vi "Register gRPC Methods.vi"(8 "error in (no error)":errorcluster, 11 "gRPC service in":refnum<class "CanReaderNixnet.lvclass">) -> (0 "error out":errorcluster, 3 "gRPC service out":refnum<class "CanReaderNixnet.lvclass">)   [LabVIEW 2021, in "CanReaderNixnet_server.lvlib" / "CanReaderNixnet.lvclass"]
uses:
  CanReaderNixnet.lvclass
  typeDefs/Server Internal UEs.ctl
  typeDefs/Server Internal Message.ctl
  typeDefs/Server gRPC UEs.ctl
  <vilib>/gRPC/LabVIEW gRPC Library/Server API/typeDefs/gRPCId Cluster.ctl
  <vilib>/gRPC/LabVIEW gRPC Library/Shared/grpcId.ctl
  CanReaderNixnet.lvclass/CanReaderNixnet.ctl
  <vilib>/gRPC/LabVIEW gRPC Library/grpc-lvsupport-release.lvlib
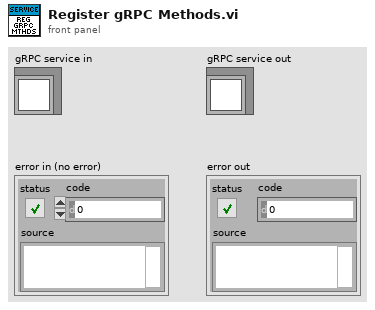
[diagram p1: front panel]
types:
  T1 = typedef "CanReaderNixnet_server.lvlib/CanReaderNixnet.lvclass/Server gRPC UEs.ctl" = cluster{"CanReaderNixnet GetDevices gRPC UE":refnum<user-event>, "CanReaderNixnet GetStatistics gRPC UE":refnum<user-event>, "CanReaderNixnet SetInterfaceBlink gRPC UE":refnum<user-event>, "CanReaderNixnet GetCANStatus gRPC UE":refnum<user-event>}
  T2 = typedef "CanReaderNixnet_server.lvlib/CanReaderNixnet.lvclass/Server Internal UEs.ctl" = cluster{"CanReaderNixnet GetDevices Internal UE":refnum<user-event>, "CanReaderNixnet GetStatistics Internal UE":refnum<user-event>, "CanReaderNixnet SetInterfaceBlink Internal UE":refnum<user-event>, "CanReaderNixnet GetCANStatus Internal UE":refnum<user-event>}
  T3 = typedef "grpc-lvsupport-release.lvlib/grpcId.ctl" = u64
  T4 = typedef "CanReaderNixnet_server.lvlib/CanReaderNixnet.lvclass/Server Internal Message UE.ctl" = refnum<user-event>
  T5 = typedef "grpc-lvsupport-release.lvlib/gRPCId Cluster UE.ctl" = refnum<user-event>
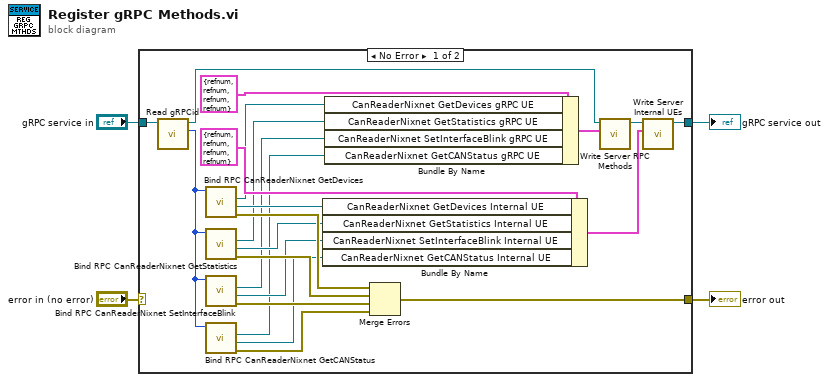
[diagram p0: block diagram]
diagram:
  n1 = case shown="No Error" "error in (no error)" {
    selector: "error in (no error)" -> [_ w27]
    tunnel: "gRPC service in" -> [w18 w28]
    tunnel: [w26 w27] -> w3
    tunnel: [w25 w28] -> w2
    frame No Error {
      n2 = call-dynamic "Read gRPCid.vi"("gRPC service in"=w18) -> ("gRPCid"=w17:T3, "gRPC service out"=w19:refnum<class "CanReaderNixnet.lvclass">)  [unwired: 8 in, 1 out]
      n3 = call "Bind RPC CanReaderNixnet GetDevices.vi"("gRPCid server in"=w17) -> ("error out"=w16:errorcluster, "CanReaderNixnet GetDevices Internal UE"=w14:T4, "CanReaderNixnet GetDevices gRPC UE"=w15:T5)  [unwired: 7 in, 1 out]
      n4 = call "Bind RPC CanReaderNixnet GetStatistics.vi"("gRPCid server in"=w17) -> ("error out"=w13:errorcluster, "CanReaderNixnet GetStatistics Internal UE"=w11:T4, "CanReaderNixnet GetStatistics gRPC UE"=w12:T5)  [unwired: 7 in, 1 out]
      n5 = call "Bind RPC CanReaderNixnet SetInterfaceBlink.vi"("gRPCid server in"=w17) -> ("error out"=w10:errorcluster, "CanReaderNixnet SetInterfaceBlink Internal UE"=w8:T4, "CanReaderNixnet SetInterfaceBlink gRPC UE"=w9:T5)  [unwired: 7 in, 1 out]
      n6 = call "Bind RPC CanReaderNixnet GetCANStatus.vi"("gRPCid server in"=w17) -> ("error out"=w7:errorcluster, "CanReaderNixnet GetCANStatus Internal UE"=w5:T4, "CanReaderNixnet GetCANStatus gRPC UE"=w6:T5)  [unwired: 7 in, 1 out]
      n7 = Bundle By Name ("Bundle Internal UEs")(cluster=T2 {"CanReaderNixnet GetDevices Internal UE"=refnum, "CanReaderNixnet GetStatistics Internal UE"=refnum, "CanReaderNixnet SetInterfaceBlink Internal UE"=refnum, "CanReaderNixnet GetCANStatus Internal UE"=refnum} ("Server Internal UEs"), "CanReaderNixnet GetDevices Internal UE"=w14, "CanReaderNixnet GetStatistics Internal UE"=w11, "CanReaderNixnet SetInterfaceBlink Internal UE"=w8, "CanReaderNixnet GetCANStatus Internal UE"=w5) -> (w24:T2)
      n8 = Bundle By Name ("Bundle gRPC UEs")(cluster=T1 {"CanReaderNixnet GetDevices gRPC UE"=refnum, "CanReaderNixnet GetStatistics gRPC UE"=refnum, "CanReaderNixnet SetInterfaceBlink gRPC UE"=refnum, "CanReaderNixnet GetCANStatus gRPC UE"=refnum} ("gRPC Server Method Events"), "CanReaderNixnet GetDevices gRPC UE"=w15, "CanReaderNixnet GetStatistics gRPC UE"=w12, "CanReaderNixnet SetInterfaceBlink gRPC UE"=w9, "CanReaderNixnet GetCANStatus gRPC UE"=w6) -> (w21:T1)
      n9 = Merge Errors(w16, w13, w10, w7) -> (w26:errorcluster)
      n10 = call "Write Server RPC Methods.vi"("Server RPC Methods"=w21, "gRPC service in"=w19) -> ("gRPC service out"=w22:refnum<class "CanReaderNixnet.lvclass">)  [unwired: 8 in, 1 out]
      n11 = call "Write Server Internal UEs.vi"("Server Internal UEs"=w24, "gRPC service in"=w22) -> ("gRPC service out"=w25:refnum<class "CanReaderNixnet.lvclass">)  [unwired: 8 in, 1 out]
    }
    frame Error {
    }
  }
  "error out" <- w3
  "gRPC service out" <- w2
